vi "uService GUI.vi"(8 "error in (no error)":errorcluster, 11 "uService Template in":refnum<class "Error Manager.lvclass">) -> (3 "uService Template out":refnum<class "Error Manager.lvclass">)   [LabVIEW 2020, in "TALOS.lvlib" / "Error Manager.lvlib" / "Error Manager.lvclass"]
uses:
  Error Manager.lvclass
  C:/LabVIEW Code/TALOS/talos/Father of all uServices/Father of all uServices/Father of all uServices.lvclass
  Error Info.ctl
  Ancestor/Ancestor/Ancestor.lvclass/Ancestor.ctl
  Support VIs/Substitute Error.vi
  Support VIs/Generate Error.vi
  FGV/Error Memory/Get Error Description.vi
  Support VIs/Get PC name.vi
  Ancestor/Ancestor/Read ID.vi
  Support VIs/Get Class Name.vi
  FGV/Error Memory/Error Memory Core.vi
  <vilib>/AdvancedString/Delimited String to 1D String Array.vi
  Support VIs/Circus Root Path.vi
  FGV/Error Memory/Error Crt Lvl checker.vi
  FGV/Error Memory/Error Memory Core.vi/40c8088d-b597-4017-91af-faa98e00292e.vi
  FGV/Error Memory/Error Memory Core.vi/d4a3ab98-063c-4e44-b43d-fbdcfe6c2be2.vi
  Father of all uServices/Father of all uServices/Father of all uServices.lvclass
  C:/LabVIEW Code/TALOS/builds/Actor Framework PPL/Actor Framework.lvlibp/1abvi3w/vi.lib/ActorFramework/Actor/Actor.lvclass
  Support VIs/Global Memory.vi
  builds/Actor Framework PPL/Actor Framework.lvlibp/1abvi3w/vi.lib/ActorFramework/Actor/Read Self Enqueuer.vi
  builds/Actor Framework PPL/Actor Framework.lvlibp/1abvi3w/vi.lib/ActorFramework/Stop Msg/Send Normal Stop.vi
  <vilib>/Utility/LVClass/Get LV Class Name.vi
  Support VIs/Is in Packed Library.vi
  Support VIs/TALOS Root path.vi
  Support VIs/Read CSV worksheet.vi
  Support VIs/Global Constants.vi
  <vilib>/Utility/error.llb/General Error Handler.vi
  Support VIs/Error Log.vi
  Ancestor/Ancestor/Ancestor.lvclass
  <vilib>/Comparison/Equal/Equal Functor/Equal Functor.lvclass
  TALOS.lvlib
panel:
  in  "Clear Filters":bool
  in  "Filter out Errors":bool
  in  "Errors to filter":i32[](array[numeric])
  in  "Suppress error pop-ups":bool
  in  "Dismiss All Errors":bool
  in  "Generate Error":bool
  in  "Error to generate":errorcluster
  in  "Dismiss Errror":bool
  out "Error Details Display":string
  in  "View Error Details":bool
  in  "Select Error":i32
  out "Array of Errors Display":T1[](array[typedef]) {"Time Stamp" format="%<%x %.3X>T"}
  in  "stop New uService":bool
  # "Error Manager"
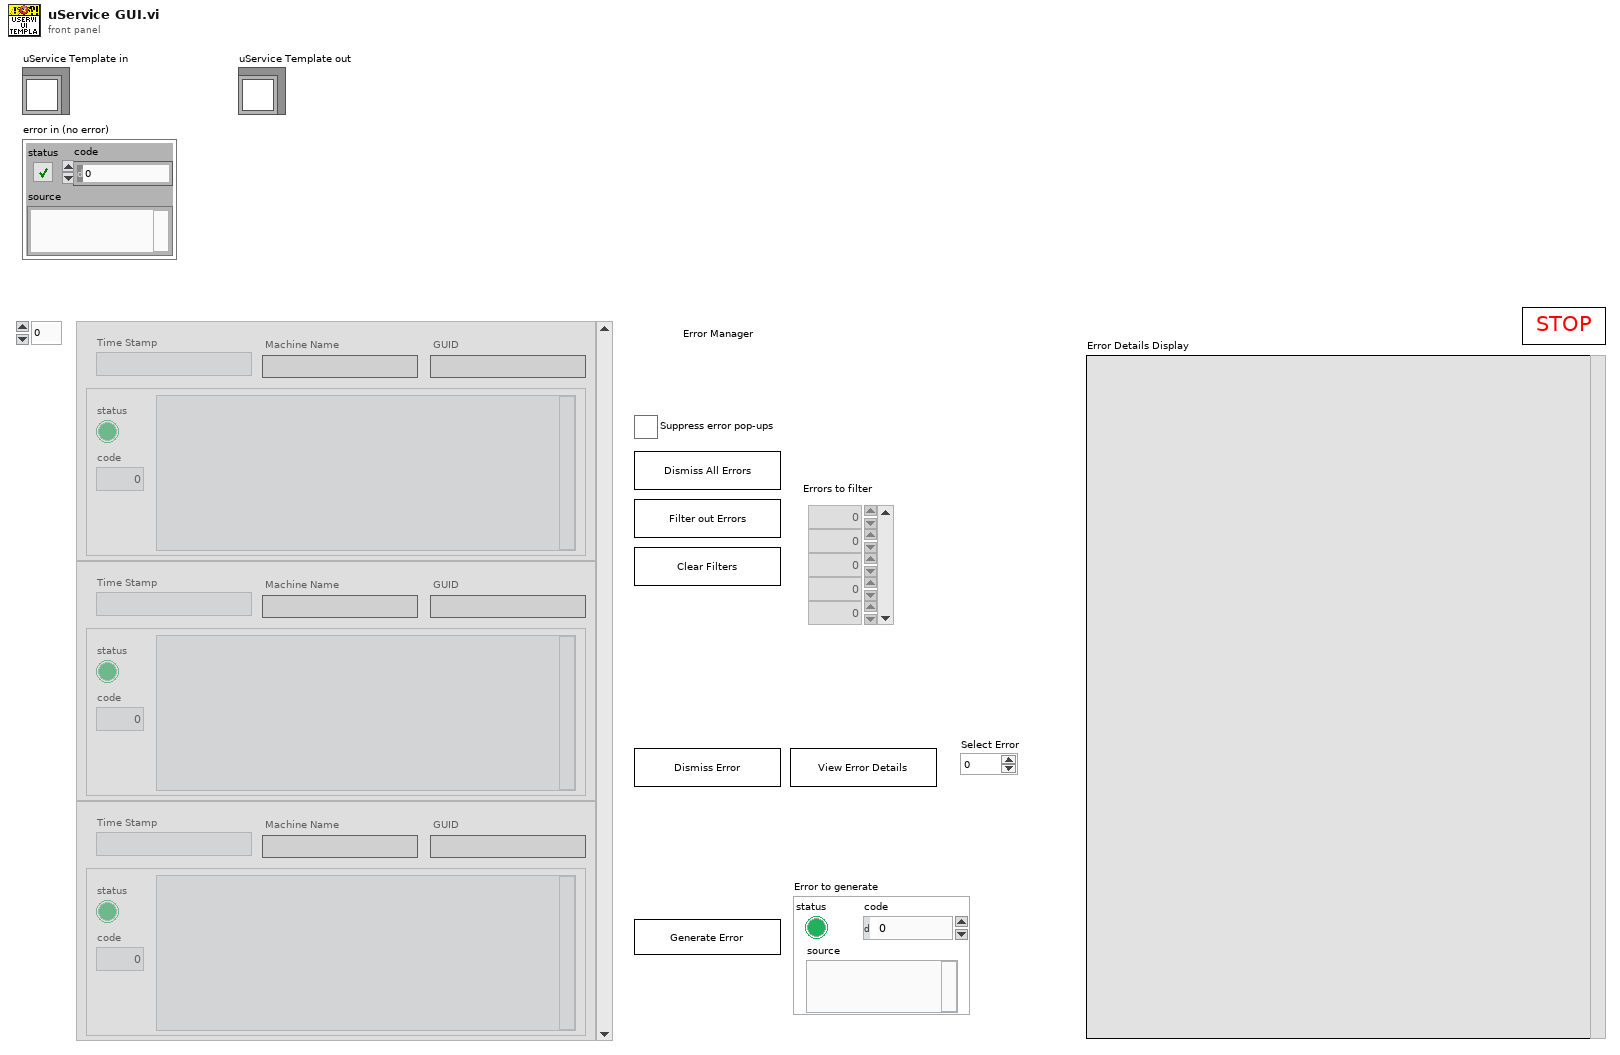
[diagram p1: front panel]
types:
  T1 = typedef "TALOS.lvlib/Error Manager.lvlib/Error Manager.lvclass/Error Info.ctl" = cluster{"error out":errorcluster, "Time Stamp":timestamp, "Machine Name":string, "GUID":string}
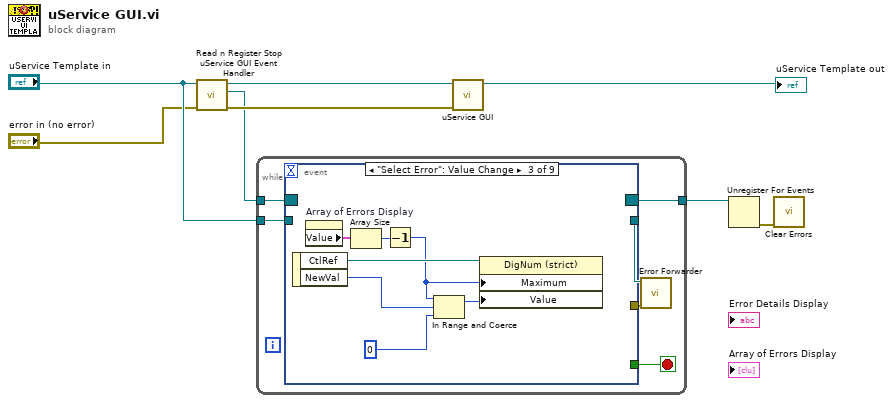
[diagram p0: block diagram]
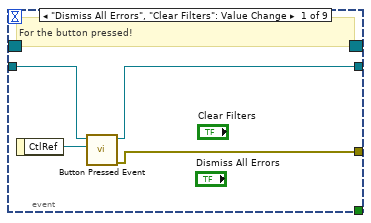
[diagram p2: hidden frame]
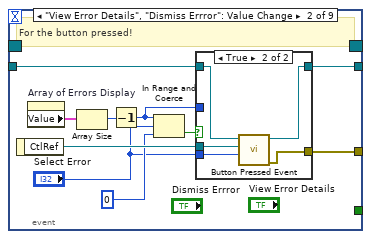
[diagram p3: hidden frame]
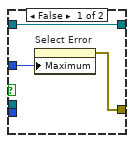
[diagram p4: hidden frame]
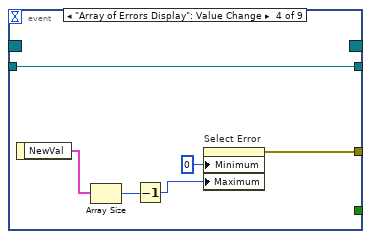
[diagram p5: hidden frame]
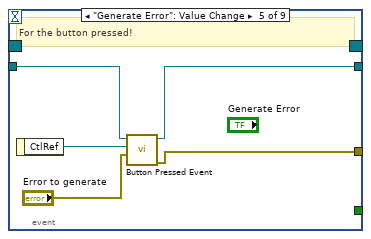
[diagram p6: hidden frame]
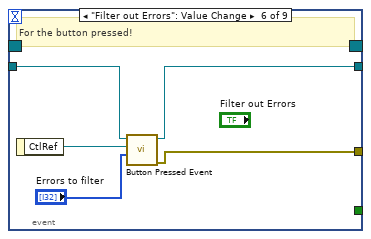
[diagram p7: hidden frame]
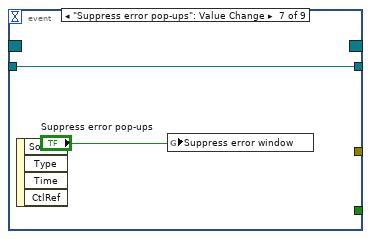
[diagram p8: hidden frame]
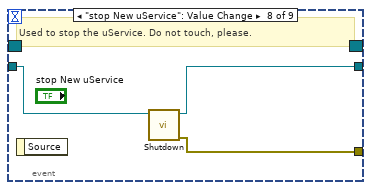
[diagram p9: hidden frame]
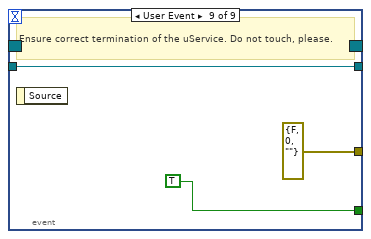
[diagram p10: hidden frame]
diagram:
  n1 = call-dynamic "Read n Register Stop uService GUI Event Handler .vi"("error in (no error)"="error in (no error)", "uService Template in"="uService Template in") -> ("error out"=w6:errorcluster, "Stop uService GUI Event Ref"=w5:refnum<event-registration>, "uService Template out"=w7:refnum<class "Error Manager.lvclass">)  [unwired: 7 in]
  n2 = while {
    tunnel: [w14] -> w8
    tunnel: w5 -> [w12]
    tunnel: "uService Template in" -> [w11]
    stop <- w13 stop-if-true
    n3 = event shown="[2] \"Select Error\": Value Change" {
      selector: w12 -> [_ _ _ _ _ _ _ _ _]
      dyn-events: [_ _ _ _ _ _ _ _ _] -> w14
      timeout: _ -> [_ _ _ _ _ _ _ _ _]
      tunnel: [_ _ _ _ _ _ _ _ TRUE] -> w13
      tunnel: w11 -> [w18 w28 _ w44 w54 w59 w60 w64 w66]
      tunnel: [w16 w22 _ w44 w52 w57 w60 w63 w66] -> w10
      tunnel: [w15 w26 _ w49 w51 w56 _ w62 errorcluster {"status"=FALSE, "code"=0, "source"=""} ("error in (no error)")] -> w9
      event "Dismiss All Errors", "Clear Filters": Value Change {
        # "For the button pressed!"
        n4 = event-data() -> ("CtlRef"=w17:refnum<vi>)  [unwired: 1 in]
        n5 = call-dynamic "Button Pressed Event.vi"("CtlRef"=w17, "uService Template in"=w18) -> ("error out"=w15:errorcluster, "uService Template out"=w16:refnum<class "Error Manager.lvclass">)  [unwired: 8 in]
      }
      event "View Error Details", "Dismiss Errror": Value Change {
        # "For the button pressed!"
        n6 = event-data() -> ("CtlRef"=w27:refnum<vi>)  [unwired: 1 in]
        n7 = property on="Array of Errors Display" class="Arr (strict)"() -> ("Value"=w25:T1[])  [unwired: 2 in, 2 out]
        n8 = Array Size(array=w25) -> (size(s)=w21:i32)
        n9 = Decrement(x=w21) -> (x-1=w20:i32)
        n10 = In Range and Coerce(upper limit=w20, x="Select Error", lower limit=0) -> (In Range?=w23:bool)  [unwired: 1 out]
        n11 = case shown="True" w23 {
          tunnel: w28 -> [w31 w34]
          tunnel: w27 -> [_ w36]
          tunnel: [w30 w35] -> w26
          tunnel: [w31 w33] -> w22
          tunnel: w20 -> [w29 _]
          tunnel: "Select Error" -> [_ w32]
          frame False {
            n12 = property on="Select Error" class="DigNum (strict)"("Maximum"=w29) -> (error out=w30:errorcluster)  [unwired: 2 in, 1 out]
          }
          frame True {
            n13 = call-dynamic "Button Pressed Event.vi"("Data"=w32, "CtlRef"=w36, "uService Template in"=w34) -> ("error out"=w35:errorcluster, "uService Template out"=w33:refnum<class "Error Manager.lvclass">)  [unwired: 7 in]
          }
        }
      }
      event "Select Error": Value Change {
        n14 = event-data() -> ("CtlRef"=w43:refnum<vi>, "NewVal"=w38:i32)  [unwired: 1 in]
        n15 = property on="Array of Errors Display" class="Arr (strict)"() -> ("Value"=w42:T1[])  [unwired: 2 in, 2 out]
        n16 = Array Size(array=w42) -> (size(s)=w41:i32)
        n17 = Decrement(x=w41) -> (x-1=w40:i32)
        n18 = In Range and Coerce(upper limit=w40, x=w38, lower limit=u32 0) -> (coerced(x)=w37:u32)  [unwired: 1 out]
        n19 = property class="DigNum (strict)"(reference=w43, "Maximum"=w40, "Value"=w37) -> ()  [unwired: 1 in, 2 out]
      }
      event "Array of Errors Display": Value Change {
        n20 = event-data() -> ("NewVal"=w48:T1[])  [unwired: 1 in]
        n21 = Array Size(array=w48) -> (size(s)=w47:i32)
        n22 = Decrement(x=w47) -> (x-1=w45:i32)
        n23 = property on="Select Error" class="DigNum (strict)"("Minimum"=0 ("Data Entry Limits:Minimum"), "Maximum"=w45) -> (error out=w49:errorcluster)  [unwired: 2 in, 1 out]
      }
      event "Generate Error": Value Change {
        # "For the button pressed!"
        n24 = event-data() -> ("CtlRef"=w53:refnum<vi>)  [unwired: 1 in]
        n25 = call-dynamic "Button Pressed Event.vi"("Data"="Error to generate", "CtlRef"=w53, "uService Template in"=w54) -> ("error out"=w51:errorcluster, "uService Template out"=w52:refnum<class "Error Manager.lvclass">)  [unwired: 7 in]
      }
      event "Filter out Errors": Value Change {
        # "For the button pressed!"
        n26 = event-data() -> ("CtlRef"=w58:refnum<vi>)  [unwired: 1 in]
        n27 = call-dynamic "Button Pressed Event.vi"("Data"="Errors to filter", "CtlRef"=w58, "uService Template in"=w59) -> ("error out"=w56:errorcluster, "uService Template out"=w57:refnum<class "Error Manager.lvclass">)  [unwired: 7 in]
      }
      event "Suppress error pop-ups": Value Change {
        n28 = event-data() -> ()  [unwired: 1 in, 4 out]
        n29 = global write "Global Memory.vi" "Suppress error window"("Suppress error pop-ups") -> ()
      }
      event "stop New uService": Value Change {
        # "Used to stop the uService. Do not touch, please."
        n30 = event-data() -> ()  [unwired: 1 in, 1 out]
        n31 = call "Shutdown.vi"("Father of all uServices in"=w64) -> ("error out"=w62:errorcluster, "Father of all uServices out"=w63:refnum<class "Error Manager.lvclass">)  [unwired: 9 in]
      }
      event User Event {
        # "Ensure correct termination of the uService. Do not touch, please."
        n32 = event-data() -> ()  [unwired: 1 in, 1 out]
      }
    }
    n33 = call "Error Forwarder.vi"("error in (no error)"=w9, "Father of all uServices in"=w10) -> ()  [unwired: 10 in]
  }
  n34 = call-parent "uService GUI.vi"("error in (no error)"=w6, "uService Template in"=w7) -> ("uService Template out"=→"uService Template out":refnum<class "Error Manager.lvclass">)  [unwired: 9 in]
  n35 = Unregister For Events(event registration refnum=w8) -> (error out=w1:errorcluster)  [unwired: 1 in]
  n36 = call <vilib>:"Clear Errors.vi"("error in (no error)"=w1) -> ()  [unwired: 5 in, 2 out]
